vi "Read type.vi"(8 "error in (no error)":errorcluster, 11 "ZM-PC-package in":refnum<class "ZM-PC-package.lvclass">) -> (0 "error out":errorcluster, 2 "ZM-PC-PACKAGE_TYPE":T1, 3 "ZM-PC-package out":refnum<class "ZM-PC-package.lvclass">)   [LabVIEW 2020, in "ZM-PC-packages.lvlib" / "ZM-PC-package.lvclass"]
doc: "Reads one field of this class's private data. Generated by lvai_create_accessors from the class private data control."
uses:
  ZM-PC-package.lvclass
  ZM-PC-package.lvclass/ZM-PC-package.ctl
  ZM-PC-PACKAGE_TYPE.ctl
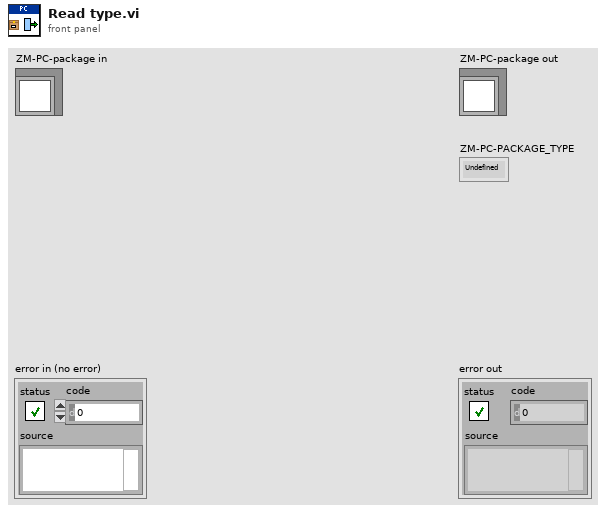
[diagram p1: front panel]
types:
  T1 = typedef "ZM-PC-packages.lvlib/ZM-PC-package.lvclass/ZM-PC-PACKAGE_TYPE.ctl" = enum16{"Undefined", "TestPackage", "ErrorPackage"}
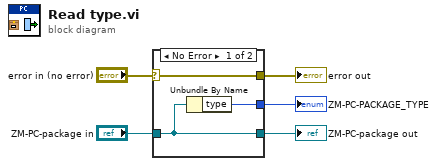
[diagram p0: block diagram]
diagram:
  n1 = case shown="No Error" "error in (no error)" {
    selector: "error in (no error)" -> [w8 w9]
    tunnel: [w8 w9] -> w4
    tunnel: [w7 w10] -> w2
    tunnel: "ZM-PC-package in" -> [w7 w10]
    tunnel: [w6 _] -> w1
    frame No Error {
      n2 = Unbundle By Name(w7) -> ("type"=w6:T1)
    }
    frame Error {
    }
  }
  "error out" <- w4
  "ZM-PC-package out" <- w2
  "ZM-PC-PACKAGE_TYPE" <- w1
